vi "Get-DIO-DAQmx-Cfg.vi"(8 "error in (no error)":errorcluster, 11 "DIO_Channel in":refnum<class "DIO_Channel.lvclass">) -> (0 "error out":errorcluster, 2 "DAQmx-Cfg":refnum<class "DIO-Configuration.lvclass">, 3 "DIO_Channel out":refnum<class "DIO_Channel.lvclass">)   [LabVIEW 2021, in "DAQmx.lvlib" / "DIO_Channel.lvclass"]
uses:
  DIO_Channel.lvclass
  C:/Users/averna/Documents/LV Gym DEMO/Factory Pattern/Device Channels/Dependencies/DIO-Channel.lvlibp/Channels/DIO-Channel/DIO_Channel_class/DIO_Channel.lvclass
  DIO-Configuration_class/DIO-Configuration.lvclass
  Dependencies/DIO-Channel.lvlibp/Channels/DIO-Channel/DIO_Channel_class/Properties/GetDIOConfiguration.vi
  Dependencies/DIO-Channel.lvlibp/Channels/DIO-Channel/DIO-Configuration_class/DIO-Configuration.lvclass
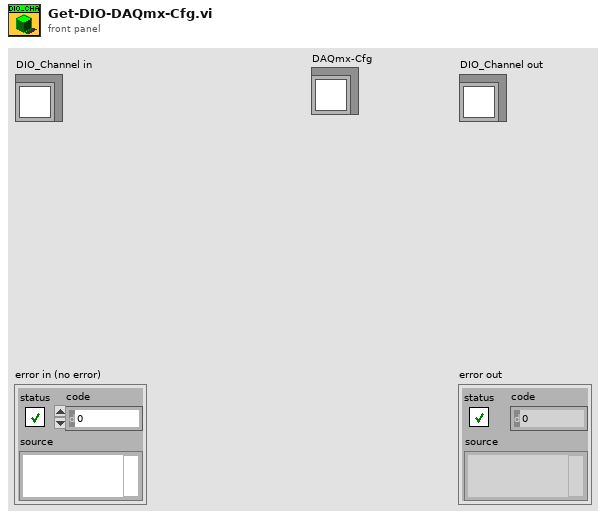
[diagram p1: front panel]
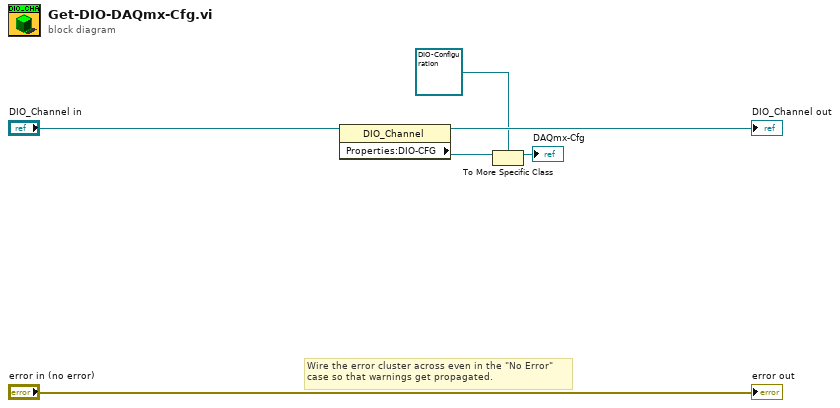
[diagram p0: block diagram]
diagram:
  # "Wire the error cluster across even in the \"No Error\"\ncase so that warnings get propagated."
  n1 = property class="DIO_Channel"(reference="DIO_Channel in") -> (reference out=→"DIO_Channel out":refnum<class "DIO_Channel.lvclass">, "Properties:DIO-CFG"=w3:refnum<class "DIO-Configuration.lvclass">)  [unwired: 1 in, 1 out]
  n2 = To More Specific Class(target class=refnum<class "DIO-Configuration.lvclass"> refnum ("DAQmx.lvlib:DIO_CFG"), reference=w3) -> (specific class reference=→"DAQmx-Cfg":refnum<class "DIO-Configuration.lvclass">)  [unwired: 1 in, 1 out]
  "error out" <- "error in (no error)"
